vi "Init UltraSonic.vi"(8 "error in (no error)":errorcluster, 11 "M5Stack UltraSonic Range Sensor in":refnum<class "M5Stack UltraSonic Range Sensor.lvclass">) -> (0 "error out":errorcluster, 3 "M5Stack UltraSonic Range Sensor out":refnum<class "M5Stack UltraSonic Range Sensor.lvclass">)   [LabVIEW 2020, in "CTI-Peripheral.lvlib" / "M5Stack UltraSonic Range Sensor.lvclass"]
uses:
  M5Stack UltraSonic Range Sensor.lvclass
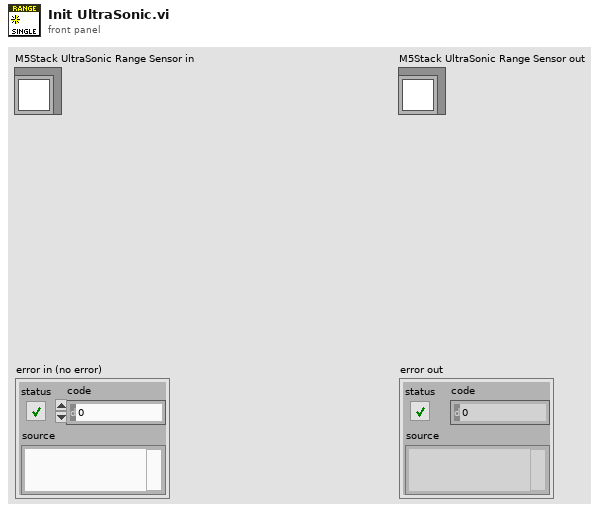
[diagram p1: front panel]
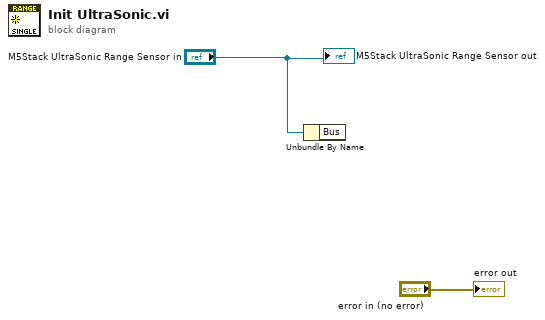
[diagram p0: block diagram]
diagram:
  n1 = Unbundle By Name("M5Stack UltraSonic Range Sensor in") -> ()  [unwired: 1 out]
  "error out" <- "error in (no error)"
  "M5Stack UltraSonic Range Sensor out" <- "M5Stack UltraSonic Range Sensor in"
